vi "Disconnect.vi"(8 "Error In":errorcluster, 10 "Description":string="Normal Shutdown", 11 "Session In":refnum<class "Session.lvclass">) -> (0 "Error Out":errorcluster, 3 "Sesssion Out":refnum<class "Session.lvclass">)   [LabVIEW 2018, in "Toolkit.lvlib" / "Session.lvclass"]
doc: "Disconnects a session from a remote SSH server. The user will need to be re-authenticated after the session is disconnected. This is typically called immediate BEFORE destroying the session. This does NOT free the underlying resource within the libssh2 shared library."
uses:
  Session.lvclass
  Session.lvclass/Session.ctl
  SSH/SSH.lvclass/SSH.ctl
  Toolkit.lvlib
  SSH/SSH.lvclass
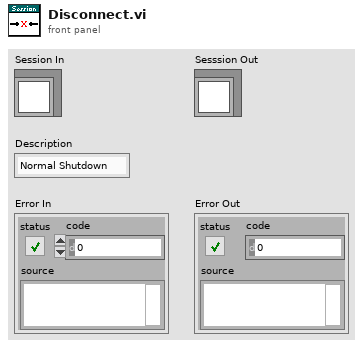
[diagram p1: front panel]
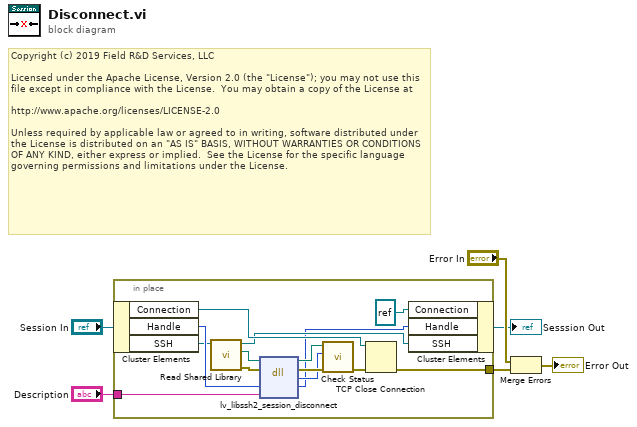
[diagram p0: block diagram]
diagram:
  # "Copyright (c) 2019 Field R&D Services, LLC\n\nLicensed under the Apache License, Version 2.0 (the \"License\"); you may not use this file except in compliance with the License.  You may obtain a copy of the License at\n\nhttp://www.apache.org/licenses/LICENSE-2.0\n\nUnless required by applicable law or agreed to in writing, software distributed under the License is distributed on an \"AS IS\" BASIS, WITHOUT WARRANTIES OR CONDITIONS OF ANY KIND, either express or implied.  See the License for the specific language governing permissions and limitations under the License."
  n1 = in-place {
    in-place-border: "Description" -> [w18]
    in-place-border: [w17] -> w1
    n2 = in-place-cluster #1("Session In") -> ("Connection"=w20:refnum<k5>, "Handle"=w16:u64, "SSH"=w11:refnum<class "SSH.lvclass">)
    n3 = call "Read Shared Library.vi"("SSH In"=w11) -> ("Error Out"=w9:errorcluster, "libssh2lv Shared Library"=w8:path, "SSH Out"=w10:refnum<class "SSH.lvclass">)  [unwired: 8 in]
    n4 = dll-call lib="libssh2lv.*" fn="lv_libssh2_session_disconnect"(path in=w8, error in=w9, "session"=w16, "description"=w18) -> (path out=w14:path, error out=w15:errorcluster, "result"=w12:i32, "session"=w7:u64)  [unwired: 2 in]
    n5 = call "Check Status.vi"("Error In"=w15, "Status"=w12, "libssh2lv Shared Library In"=w14) -> ("Error Out"=w13:errorcluster)  [unwired: 7 in, 1 out]
    n6 = TCP Close Connection(connection ID=w20, error in (no error)=w13) -> (error out=w17:errorcluster)  [unwired: 1 in, 1 out]
    n7 = in-place-cluster #1("Connection"=refnum<k5> refnum, "Handle"=w7, "SSH"=w10) -> (→"Sesssion Out":refnum<class "Session.lvclass">)
  }
  n8 = Merge Errors("Error In", w1) -> (→"Error Out":errorcluster)
